vi "numCmd_Recv_Array.vi"(7 "Command Name":string, 11 "Initial Values":dbl[](array[numeric])) -> (0 "error out":errorcluster, 2 "Any Changed":bool, 3 "Values":dbl[](array[numeric]))   [LabVIEW 2019, in "Trajectory_Library.lvlib"]
uses:
  Trajectory_Library.lvlib
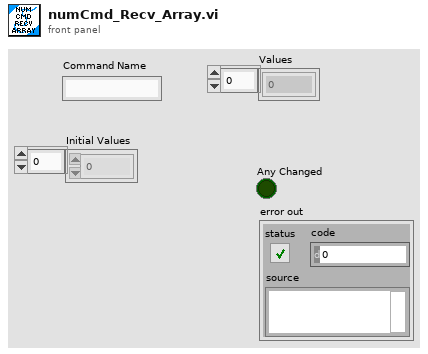
[diagram p1: front panel]
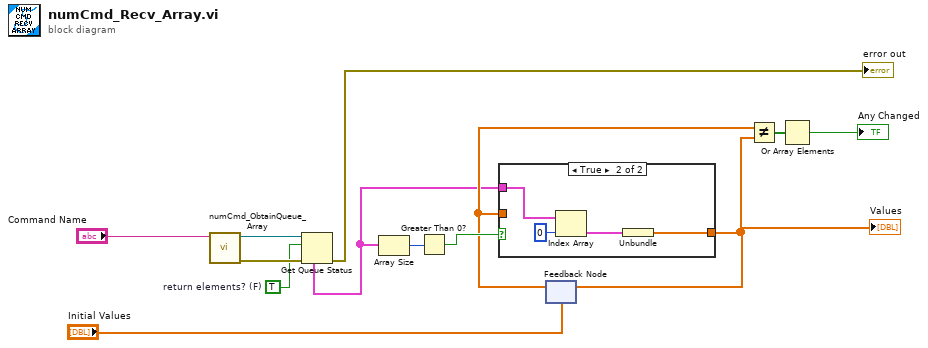
[diagram p0: block diagram]
diagram:
  w9 = TRUE  # return elements? (F)
  n1 = call "numCmd_ObtainQueue_Array.vi"("Command Name"="Command Name") -> ("error out"=w13:errorcluster, "queue out"=w2:refnum<queue>)  [unwired: 9 in]
  n2 = Get Queue Status(queue=w2, return elements? (F)=w9, error in (no error)=w13) -> (error out=→"error out":errorcluster, elements=w1:cluster{dbl[]}[])  [unwired: 6 out]
  n3 = Array Size(array=w1) -> (size(s)=w12:i32)
  n4 = Greater Than 0?(x=w12) -> (x > 0?=w11:bool)
  n5 = feedback #1("Initial Values") -> (w10:dbl[])
  n6 = case shown="True" w11 {
    tunnel: [w14 w15] -> w5
    tunnel: w10 -> [w14 _]
    tunnel: w1 -> [_ w17]
    frame False {
    }
    frame True {
      n7 = Index Array(array=w17, index=0) -> (element=w16:cluster{dbl[]})
      n8 = Unbundle(w16) -> (w15:dbl[])
    }
  }
  "Values" <- w5
  n9 = feedback-in #1(w5) -> ()
  n10 = Not Equal?(x=w10, y=w5) -> (x != y?=w4:bool[])
  n11 = Or Array Elements(Boolean array=w4) -> (logical OR=→"Any Changed":bool)
